vi "Start Test.vi"(8 "error in (no error)":errorcluster, 10 "Tests":string[](array[string]), 11 "XML Report In":refnum<class "XML Report.lvclass">) -> (0 "error out":errorcluster, 3 "XML Report Out":refnum<class "XML Report.lvclass">)   [LabVIEW 2020, in "XML Report.lvclass"]
uses:
  XML Report.lvclass
  C:/git/astemes-lunit/source/Framework/Report Plugin/Report Plugin.lvclass
  Core/Result/Result.ctl
  Core/Result/Status.ctl
  Core/Result/Type.ctl
  XML Report.lvclass/XML Report.ctl
  <vilib>/xml/NI_XML.lvlib
  <resource>/objmgr/DOMUserDefRef.rc
  Core/Result/Result.lvlib
  Framework/Report Plugin/Report Plugin.lvclass
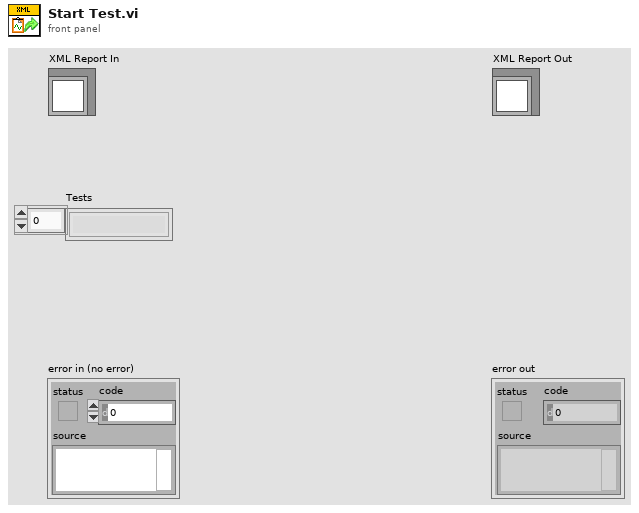
[diagram p1: front panel]
types:
  T1 = typedef "Result.lvlib/Result.ctl" = cluster{"Name":string, "Description":string, "Status":T2, "Result Type":T3, "Execution Time":dbl, "Data":cluster{"Expected":variant, "Actual":variant, "Delta":variant}}
  T2 = typedef "Result.lvlib/Status.ctl" = enum16{"", "Passed", "Failed", "Error", "Skipped", "Setup Error", "Broken", "Teardown Error"}
  T3 = typedef "Result.lvlib/Type.ctl" = enum16{"Test Case", "Test Suite", "Test Run", "Pass", "Fail", "Skip", "Pass if", "Fail if", "Pass if Error", "Fail if Error", "Pass if Equal", "Fail if Equal"}
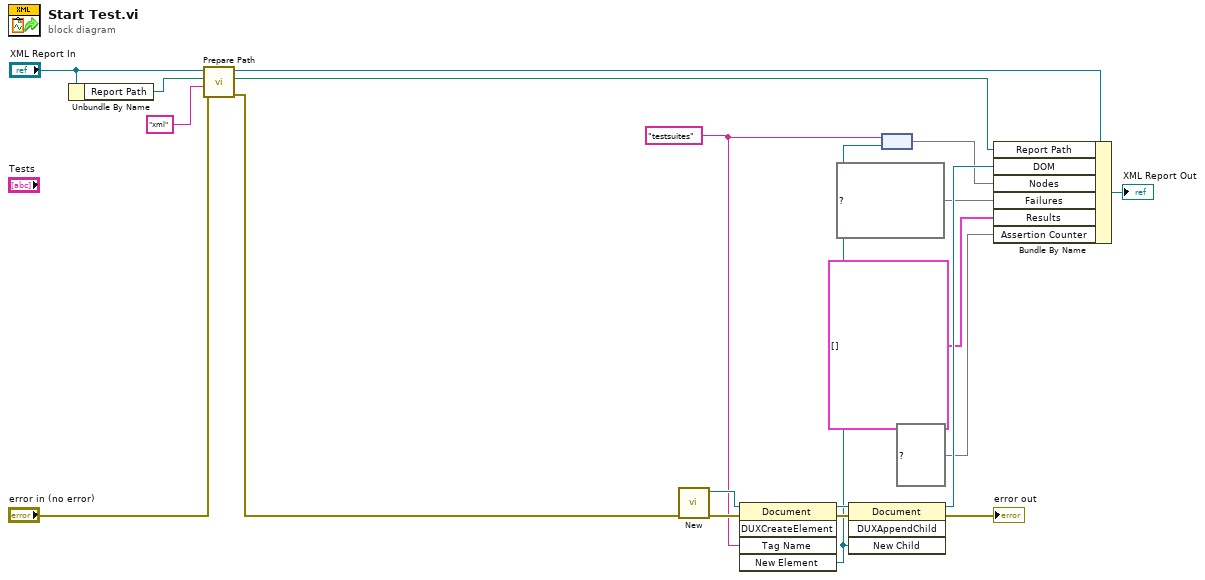
[diagram p0: block diagram]
diagram:
  w13 = "testsuites" ("Tag Name")
  n1 = Unbundle By Name("XML Report In") -> ("Report Path"=w7:path)
  n2 = call "Prepare Path.vi"("error in (no error)"="error in (no error)", "Extenssion"="xml", "File Path in"=w7, "Plugin In"="XML Report In") -> ("error out"=w2:errorcluster, "Modified Path"=w6:path, "Plugin Out"=w4:refnum<class "XML Report.lvclass">)  [unwired: 5 in]
  n3 = call <vilib>:"New.vi"("error in (no error)"=w2) -> ("error out"=w16:errorcluster, "DOM document out"=w19:refnum<k20>)  [unwired: 7 in]
  n4 = invoke class="Document" method="DUXCreateElement"(reference=w19, error in=w16, "Tag Name"=w13) -> (reference out=w18:refnum<k20>, error out=w17:errorcluster, "New Element"=w12:refnum<k20>)  [unwired: 2 in, 2 out]
  n5 = invoke class="Document" method="DUXAppendChild"(reference=w18, error in=w17, "New Child"=w12) -> (reference out=w14:refnum<k20>, error out=→"error out":errorcluster)  [unwired: 1 in, 2 out]
  n6 = node(w13, w12) -> (w11:map{string, refnum<k20>})
  n7 = Bundle By Name(cluster=w4, "Report Path"=w6, "DOM"=w14, "Nodes"=w11, "Failures"=map{string, refnum<k20>[]} {}, "Results"=T1[] [], "Assertion Counter"=map{string, i32} {}) -> (→"XML Report Out":refnum<class "XML Report.lvclass">)
